vi "Voltage - Continuous Input00.vi"() -> ()   [LabVIEW 2017]
doc: "该范例演示了如何使用DAQmx设备进行连续带缓冲的电压测量。\n\n关于如何连接信号至DAQ设备，请查阅设备手册。"
uses:
  <vilib>/Utility/error.llb/DialogType.ctl
  <vilib>/DAQmx/read.llb/DAQmx Read (Analog 1D Wfm NChan NSamp).vi
  <vilib>/DAQmx/create/channels.llb/DAQmx Create Channel (AI-Voltage-Basic).vi
  <vilib>/DAQmx/configure/timing.llb/DAQmx Timing (Sample Clock).vi
  <vilib>/DAQmx/configure/task.llb/DAQmx Configure Logging (TDMS).vi
  <vilib>/DAQmx/configure/trigger.llb/DAQmx Start Trigger (Digital Edge).vi
  <vilib>/DAQmx/configure/trigger.llb/DAQmx Start Trigger (Analog Edge).vi
  <vilib>/DAQmx/miscellaneous.llb/DAQmx Fill In Error Info.vi
  <resource>/objmgr/daqmx.rc
  <vilib>/ptbypt/NI_PtbyPt.lvlib
panel:
  out "mean":dbl caption="均值" format="%0.2f"
  out "min value":dbl caption="最小值" format="%0.2f"
  out "x-y":dbl
  in  "触发类型":T1(tab)
  in  "数字开始参考触发边沿":i32(ring)=10280 caption="边沿" items=["上升"=10280, "下降"=10171]
  in  "数字开始参考触发源":tag="/Dev1/PFI0" caption="源"
  in  "数字暂停触发暂停条件":i32(ring)=10192 caption="暂停条件" items=["高"=10192, "低"=10214]
  in  "数字暂停参考触发源":tag="/Dev1/PFI0" caption="源"
  in  "模拟开始触发基准":dbl caption="基准" format="%0.2f"
  in  "模拟开始触发滞后":dbl caption="滞后" format="%.2f"
  in  "模拟开始触发斜坡":i32(ring)=10280 caption="斜坡" items=["上升"=10280, "下降"=10171]
  in  "模拟开始触发源":string="APFI0" caption="源"
  in  "模拟暂停触发源":string="APFI0" caption="源"
  in  "模拟暂停触发暂停条件":i32(ring)=10093 caption="暂停条件" items=["高于基准"=10093, "低于基准"=10107]
  in  "模拟暂停触发基准":dbl caption="基准" format="%.2f"
  in  "停止":bool
  out "波形图":waveform(dbl)[](graph)
  in  "TDMS文件路径":path
  in  "采样数":i32=100
  in  "采样率":dbl=1000.0
  in  "采样时钟源":tag="OnboardClock"
  in  "接线端配置":i32(ring)=-1 items=["默认"=-1, "RSE"=10083, "NRSE"=10078, "差分"=10106, "伪差分"=12529]
  in  "最大电压":dbl=5.0
  in  "最小电压":dbl=-5.0
  in  "物理通道":tag="Dev1/ai0"
  out "实际采样率":dbl=1000.0 format="%0.2f"
  in  "记录模式":i32(ring)=10231 items=["关"=10231, "记录并读取"=15842]
  # "通道设置"
  # "采集数据"
  # "定时设置"
  # "触发设置"
  # "记录设置"
  # "要启用触发，选择上面的选项卡进行配置。\n\n有些硬件只支持部分触发类型。详细信息见设备的说明文档。"
  # "连续采样定时不支持该触发类型。\n\n关于设备支持的触发源的信息，见设备说明文档。"
  # "连续采样定时不支持该触发类型。\n\n关于设备支持的触发源的信息，见设备说明文档。"
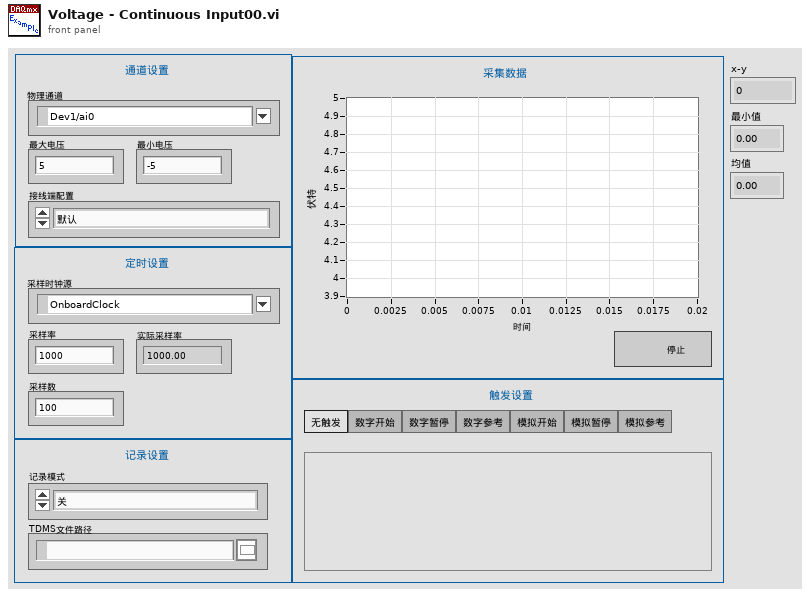
[diagram p1: front panel]
types:
  T1 = enum32{"No Trigger", "Digital Start", "Digital Pause", "Digital Reference", "Analog Start", "Analog Pause", "Analog Reference"}
  T2 = typedef "DialogType.ctl" = u16
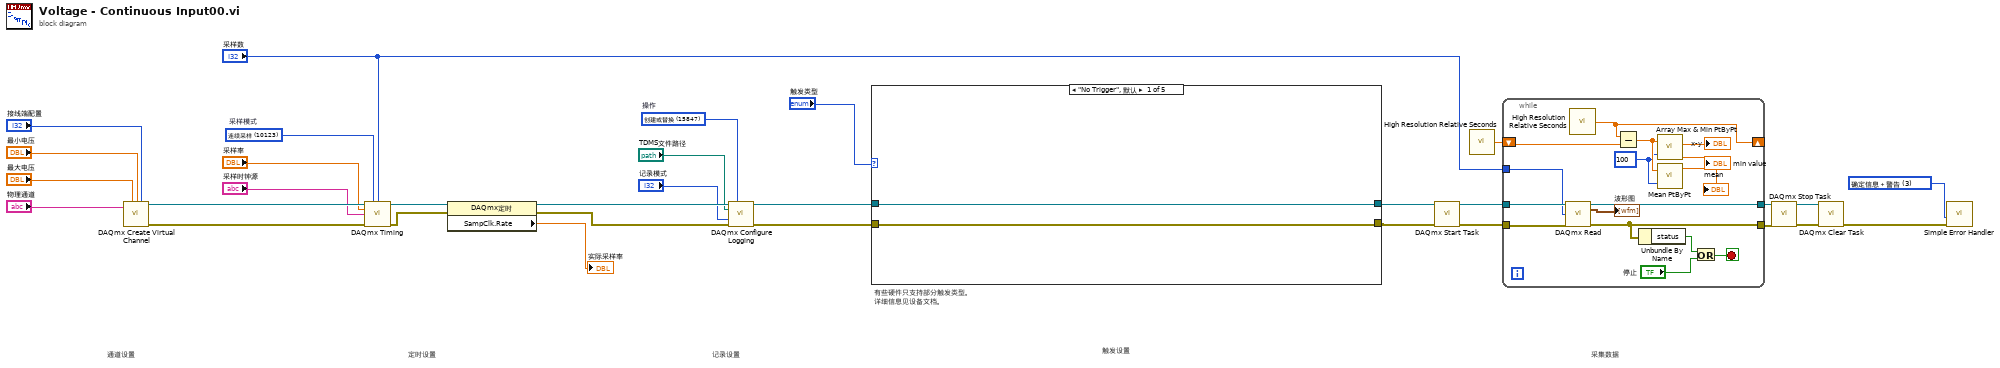
[diagram p0: block diagram]
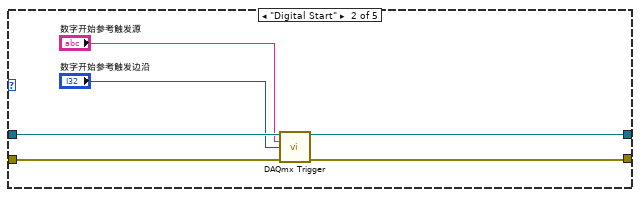
[diagram p2: hidden frame]
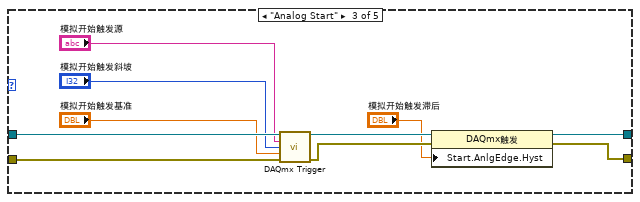
[diagram p3: hidden frame]
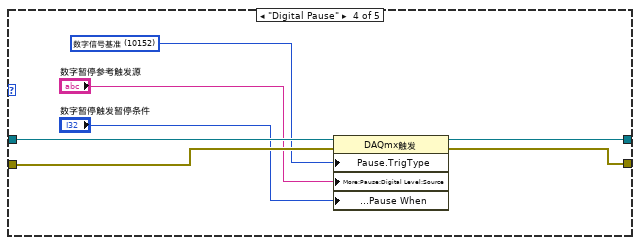
[diagram p4: hidden frame]
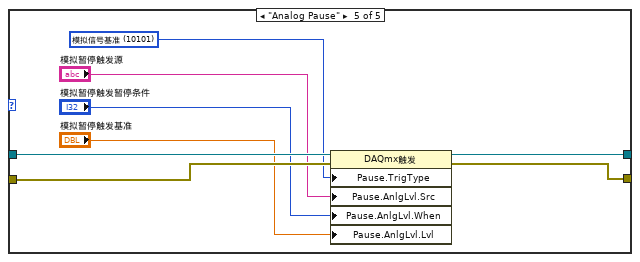
[diagram p5: hidden frame]
diagram:
  w7 = T2 3 items=["无对话框", "确定信息", "继续或停止信息", "确定信息＋警告", "继续/停止＋警告"] ("对话框类型（确定信息：1）")
  w25 = 15847 items=["打开"=10437, "打开或创建"=15846, "创建或替换"=15847, "创建"=15848]  # 操作
  w30 = 10123 items=["有限采样"=10178, "连续采样"=10123, "硬件定时单点"=12522]  # 采样模式
  # "触发设置"
  # "有些硬件只支持部分触发类型。\n详细信息见设备文档。"
  # "采集数据"
  # "定时设置"
  # "通道设置"
  # "记录设置"
  n1 = call-poly <vilib>:"DAQmx Create Virtual Channel.vi"("maximum value"="最大电压", "minimum value"="最小电压", "input terminal configuration"="接线端配置", "physical channels"="物理通道") -> ("task out"=w28:refnum<k21>, "error out"=w29:errorcluster)  [unwired: 10 in]
  n2 = call-poly <vilib>:"DAQmx Timing.vi"("task/channels in"=w28, "sample mode"=w30, "samples per channel"="采样数", "rate"="采样率", "source"="采样时钟源", "error in"=w29) -> ("task out"=w32:refnum<k21>, "error out"=w31:errorcluster)  [unwired: 8 in]
  n3 = property class="DAQmx定时"(reference=w32, error in=w31) -> (reference out=w27:refnum<k21>, error out=w26:errorcluster, "SampClk.Rate"=→"实际采样率":dbl)
  n4 = call-poly <vilib>:"DAQmx Configure Logging.vi"("task/channels in"=w27, "operation"=w25, "file path"="TDMS文件路径", "logging mode"="记录模式", "error in"=w26) -> ("task out"=w5:refnum<k21>, "error out"=w4:errorcluster)  [unwired: 9 in]
  n5 = case shown="\"No Trigger\", 默认" "触发类型" {
    tunnel: w5 -> [w34 w40 w50 w57 w65]
    tunnel: w4 -> [w33 w39 w49 w54 w62]
    tunnel: [w34 w38 w47 w56 w64] -> w2
    tunnel: [w33 w37 w46 w55 w63] -> w3
    frame "No Trigger", Default {
    }
    frame "Digital Start" {
      n6 = call-poly <vilib>:"DAQmx Trigger.vi"("task/channels in"=w40, "source"="数字开始参考触发源", "edge"="数字开始参考触发边沿", "error in"=w39) -> ("task out"=w38:refnum<k21>, "error out"=w37:errorcluster)  [unwired: 10 in]
    }
    frame "Analog Start" {
      n7 = call-poly <vilib>:"DAQmx Trigger.vi"("task/channels in"=w50, "source"="模拟开始触发源", "slope"="模拟开始触发斜坡", "level"="模拟开始触发基准", "error in"=w49) -> ("task out"=w45:refnum<k21>, "error out"=w44:errorcluster)  [unwired: 9 in]
      n8 = property class="DAQmx触发"(reference=w45, error in=w44, "Start.AnlgEdge.Hyst"="模拟开始触发滞后") -> (reference out=w47:refnum<k21>, error out=w46:errorcluster)
    }
    frame "Digital Pause" {
      w53 = 10152 items=["模拟信号基准"=10101, "模拟窗"=10103, "数字信号基准"=10152, "数字模式"=10398, "无"=10230] ("暂停.触发类型")
      n9 = property class="DAQmx触发"(reference=w57, error in=w54, "Pause.TrigType"=w53, "More:Pause:Digital Level:Source"="数字暂停参考触发源", "More:Pause:Digital Level:Pause When"="数字暂停触发暂停条件") -> (reference out=w56:refnum<k21>, error out=w55:errorcluster)
    }
    frame "Analog Pause" {
      w61 = 10101 items=["模拟信号基准"=10101, "模拟窗"=10103, "数字信号基准"=10152, "数字模式"=10398, "无"=10230] ("暂停.触发类型")
      n10 = property class="DAQmx触发"(reference=w65, error in=w62, "Pause.TrigType"=w61, "Pause.AnlgLvl.Src"="模拟暂停触发源", "Pause.AnlgLvl.When"="模拟暂停触发暂停条件", "Pause.AnlgLvl.Lvl"="模拟暂停触发基准") -> (reference out=w64:refnum<k21>, error out=w63:errorcluster)
    }
  }
  n11 = call <vilib>:"DAQmx Start Task.vi"("task/channels in"=w2, "error in"=w3) -> ("task out"=w24:refnum<k21>, "error out"=w23:errorcluster)  [unwired: 12 in]
  n12 = call <vilib>:"High Resolution Relative Seconds.vi"() -> ("relative seconds"=w1:dbl)
  n13 = while {
    tunnel: w24 -> [w81]
    tunnel: w23 -> [w80]
    tunnel: [w79] -> w11
    tunnel: [w76] -> w10
    tunnel: "采样数" -> [w73]
    shift-right: [w70] -> _
    shift-left: w1 -> [w72]
    stop <- w74 stop-if-true
    w67 = 100 ("sample length")
    n14 = call-poly <vilib>:"DAQmx Read.vi"("task/channels in"=w81, "number of samples per channel"=w73, "error in"=w80) -> ("task out"=w79:refnum<k21>, "data"=→"波形图":waveform(dbl)[], "error out"=w76:errorcluster)  [unwired: 10 in]
    n15 = call <vilib>:"High Resolution Relative Seconds.vi"() -> ("relative seconds"=w70:dbl)
    n16 = Subtract(x=w70, y=w72) -> (x-y=w68:dbl)
    n17 = Unbundle By Name(w76) -> ("status"=w75:bool)
    n18 = call <vilib>:"Array Max & Min PtByPt.vi"("input data point"=w68, "sample length"=w67) -> ("max value"=→"x-y":dbl, "min value"=→"min value":dbl)  [unwired: 1 in, 3 out]
    n19 = call <vilib>:"Mean PtByPt.vi"("x"=w68, "sample length"=w67) -> ("mean"=→"mean":dbl)  [unwired: 2 in, 1 out]
    n20 = Or(x=w75, y="停止") -> (x .or. y?=w74:bool)
  }
  n21 = call <vilib>:"DAQmx Stop Task.vi"("task/channels in"=w11, "error in"=w10) -> ("task out"=w8:refnum<k21>, "error out"=w9:errorcluster)  [unwired: 12 in]
  n22 = call <vilib>:"DAQmx Clear Task.vi"("task in"=w8, "error in"=w9) -> ("error out"=w22:errorcluster)  [unwired: 13 in]
  n23 = call <vilib>:"Simple Error Handler.vi"("type of dialog (OK msg:1)"=w7, "error in (no error)"=w22) -> ()  [unwired: 3 in, 5 out]
